vi "Write Binary Config.vi"(4 "Include Class Name":bool, 6 "byte order (0:big-endian, network order)":T1(ring), 8 "error in (no error)":errorcluster, 11 "Concatenate_STR in":refnum<class "Concatenate_STR.lvclass">) -> (0 "error out":errorcluster, 2 "Binary":string, 3 "Concatenate_STR out":refnum<class "Concatenate_STR.lvclass">)   [LabVIEW 2021, in "Concatenate_STR.lvclass"]
uses:
  <vilib>/Utility/LVClass/Get LV Class Name.vi
  Concatenate_STR.lvclass
  Concatenate_STR.lvclass/Concatenate_STR.ctl
  Abs_Types/String/Abs_String.lvclass
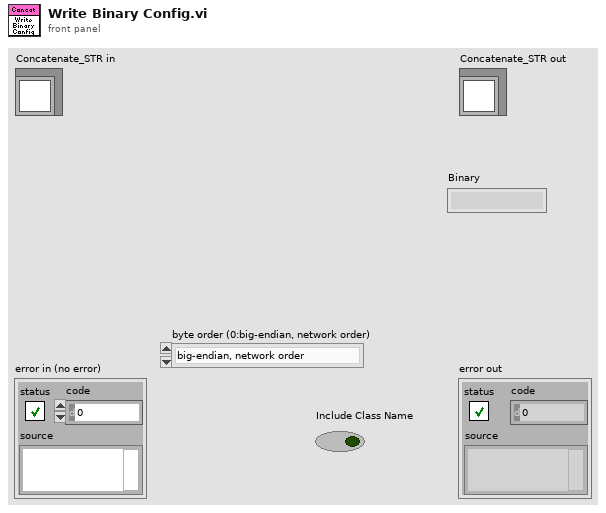
[diagram p1: front panel]
types:
  T1 = enum16{"big-endian, network order", "native, host order", "little-endian"}
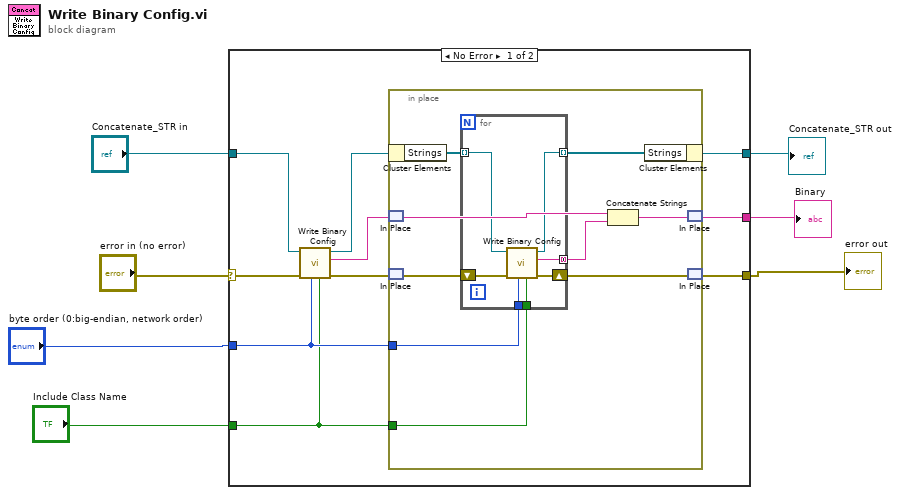
[diagram p0: block diagram]
diagram:
  n1 = case shown="No Error" "error in (no error)" {
    selector: "error in (no error)" -> [w17 w34]
    tunnel: "Concatenate_STR in" -> [w16 w35]
    tunnel: [w12 _] -> w3
    tunnel: "byte order (0:big-endian, network order)" -> [w11 _]
    tunnel: "Include Class Name" -> [w10 _]
    tunnel: [w9 w34] -> w2
    tunnel: [w8 w35] -> w1
    frame No Error {
      n2 = call-parent "Write Binary Config.vi"("Include Class Name"=w10, "byte order (0:big-endian, network order)"=w11, "error in (no error)"=w17, "Abs_Type in"=w16) -> ("error out"=w14:errorcluster, "Binary"=w13:string, "Abs_Type out"=w15:refnum<class "Concatenate_STR.lvclass">)  [unwired: 5 in]
      n3 = in-place {
        in-place-border: w11 -> [w21]
        in-place-border: w10 -> [w23]
        n4 = in-place-cluster #1(w15) -> ("Strings"=w24:refnum<class "Abs_String.lvclass">[])
        n5 = in-place-match #2(w13) -> (w20:string)
        n6 = in-place-match #3(w14) -> (w26:errorcluster)
        n7 = for {
          tunnel: [w32] -> w25 mode=indexing
          tunnel: w24 -> [w31] mode=indexing
          tunnel: w23 -> [w30]
          tunnel: w21 -> [w28]
          tunnel: [w27] -> w19 mode=concatenating
          shift-right: [w29] -> w22
          shift-left: w26 -> [w33]
          n8 = call-dynamic "Write Binary Config.vi"("Include Class Name"=w30, "byte order (0:big-endian, network order)"=w28, "error in (no error)"=w33, "Abs_Type in"=w31) -> ("error out"=w29:errorcluster, "Binary"=w27:string, "Abs_Type out"=w32:refnum<class "Abs_String.lvclass">)  [unwired: 5 in]
        }
        n9 = Concatenate Strings(w20, w19) -> (w18:string)
        n10 = in-place-cluster #1("Strings"=w25) -> (w8:refnum<class "Concatenate_STR.lvclass">)
        n11 = in-place-match #2(w18) -> (w12:string)
        n12 = in-place-match #3(w22) -> (w9:errorcluster)
      }
    }
    frame Error {
    }
  }
  "error out" <- w2
  "Concatenate_STR out" <- w1
  "Binary" <- w3
